vi "exec ui.vi"() -> ()   [LabVIEW 2013, in "execution settings.lvclass"]
uses:
  execution settings.lvclass
  <vilib>/NI/Configuration Framework/Node/NodeRef.ctl
  <vilib>/NI/Configuration Framework/Node/NISE_CEF_Node.lvclass
  <vilib>/NI/AMC/Message Queue.ctl
  <vilib>/NI/AMC/Message.ctl
  <vilib>/NI/Tools/Keyed Array/KeyedArray.ctl
  <vilib>/NI/Configuration Framework/Node/UserEventRef.ctl
  <vilib>/NI/Configuration Framework/Controls/EventCluster.ctl
  execution settings.lvclass/execution settings.ctl
  Read allow debugging.vi
  Read auto error handling.vi
  Read Is Reentrant.vi
  Read Reentrancy Type.vi
  <vilib>/NI/Tools/Keyed Array/Tools_KeyedArray.lvlib
  <vilib>/NI/AMC/AMC.lvlib
  <vilib>/NI/Configuration Framework/NISE_CEF_TreeControl.lvlib
panel:
  in  "user event":T1
  in  "main queue":T2
  in  "node ref":T3
  in  "Reentrancy Type":T4(ring)
  in  "Is Reentrant":bool
  in  "allow debugging":bool
  in  "auto error handling":bool
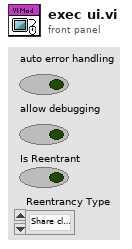
[diagram p1: front panel]
types:
  T1 = typedef "NISE_CEF_Node.lvclass/UserEventRef.ctl" = refnum<user-event>
  T2 = typedef "AMC.lvlib/Message Queue.ctl" = refnum<queue>
  T3 = typedef "NISE_CEF_Node.lvclass/NodeRef.ctl" = refnum<data-value>
  T4 = enum16{"Share clones between instances", "Preallocate clone for each instance"}
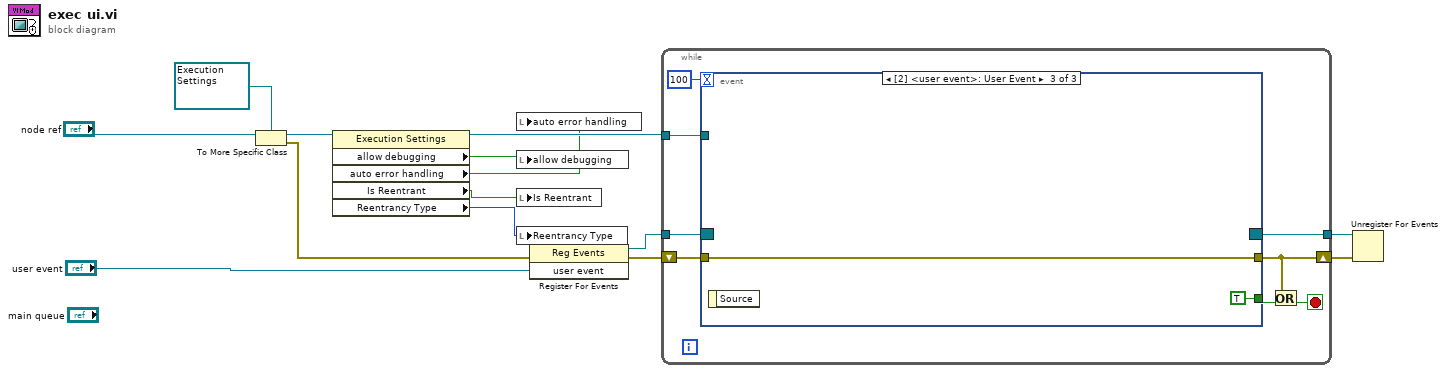
[diagram p0: block diagram]
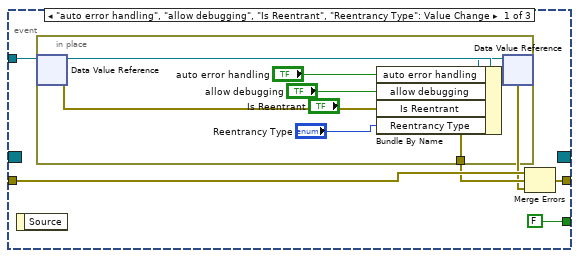
[diagram p2: hidden frame]
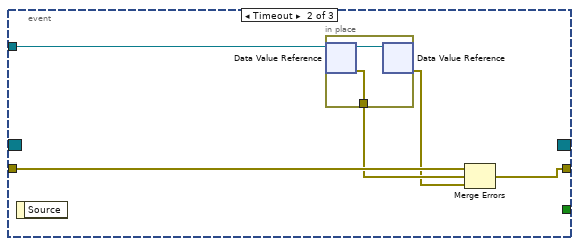
[diagram p3: hidden frame]
diagram:
  n1 = To More Specific Class(target class=refnum<data-value> refnum, reference="node ref") -> (specific class reference=w10:refnum<data-value>, error out=w8:errorcluster)  [unwired: 1 in]
  n2 = property class="Execution Settings"(reference=w10) -> (reference out=w7:refnum<data-value>, "allow debugging"=w6:bool, "auto error handling"=w5:bool, "Is Reentrant"=w4:bool, "Reentrancy Type"=w3:T4)  [unwired: 1 in, 1 out]
  n3 = local write "auto error handling"(w5) -> ()
  n4 = local write "allow debugging"(w6) -> ()
  n5 = local write "Is Reentrant"(w4) -> ()
  n6 = local write "Reentrancy Type"(w3) -> ()
  n7 = register-events(error in=w8, "user event") -> (reference out=w13:refnum<event-registration>, error out=w14:errorcluster)  [unwired: 1 in]
  n8 = while {
    shift-right: [w15] -> w12
    shift-left: w14 -> [w19]
    tunnel: w13 -> [w22]
    tunnel: [w21] -> w11
    tunnel: w7 -> [w18]
    stop <- w16 stop-if-true
    n9 = event shown="[2] <user event>: User Event" {
      selector: w22 -> [_ _ _]
      dyn-events: [_ _ _] -> w21
      timeout: 100 -> [_ _ _]
      tunnel: [FALSE _ TRUE] -> w20
      tunnel: [w26 w38 w44] -> w15
      tunnel: w19 -> [w28 w39 w44]
      tunnel: w18 -> [w27 w40 _]
      event "auto error handling", "allow debugging", "Is Reentrant", "Reentrancy Type": Value Change {
        n10 = event-data() -> ()  [unwired: 1 in, 1 out]
        n11 = in-place {
          in-place-border: [w33] -> w24
          n12 = in-place-dvr #1(w27) -> (w35:refnum<class "execution settings.lvclass">, w33:errorcluster)
          n13 = Bundle By Name(cluster=w35, "auto error handling"="auto error handling", "allow debugging"="allow debugging", "Is Reentrant"="Is Reentrant", "Reentrancy Type"="Reentrancy Type") -> (w34:refnum<class "execution settings.lvclass">)
          n14 = in-place-dvr #1(w34) -> (w23:errorcluster)  [unwired: 1 out]
        }
        n15 = Merge Errors(w28, w24, w23) -> (w26:errorcluster)
      }
      event Timeout {
        n16 = event-data() -> ()  [unwired: 1 in, 1 out]
        n17 = in-place {
          in-place-border: [w41] -> w37
          n18 = in-place-dvr #2(w40) -> (w42:refnum<class "execution settings.lvclass">, w41:errorcluster)
          n19 = in-place-dvr #2(w42) -> (w36:errorcluster)  [unwired: 1 out]
        }
        n20 = Merge Errors(w39, w37, w36) -> (w38:errorcluster)
      }
      event User Event {
        n21 = event-data() -> ()  [unwired: 1 in, 1 out]
      }
    }
    n22 = Or(x=w15, y=w20) -> (x .or. y?=w16:bool)
  }
  n23 = Unregister For Events(event registration refnum=w11, error in=w12) -> ()  [unwired: 1 out]
